vi "RemoteVI App Live Data.vi"() -> ()   [LabVIEW 2020]
doc: "Screen Live Data of RemoteVI Application Example.vi: four simulated channels on the graph Live Data (500 samples each, a new block every 100 ms), their maximum and minimum in Statistics. Pause holds the picture. Runs until the notifier RemoteVI Application Example fires (the main VI quits)."
panel:
  out "Statistics":string[][](table)
  out "Live Data":dbl[][](graph)
  in  "Pause":bool
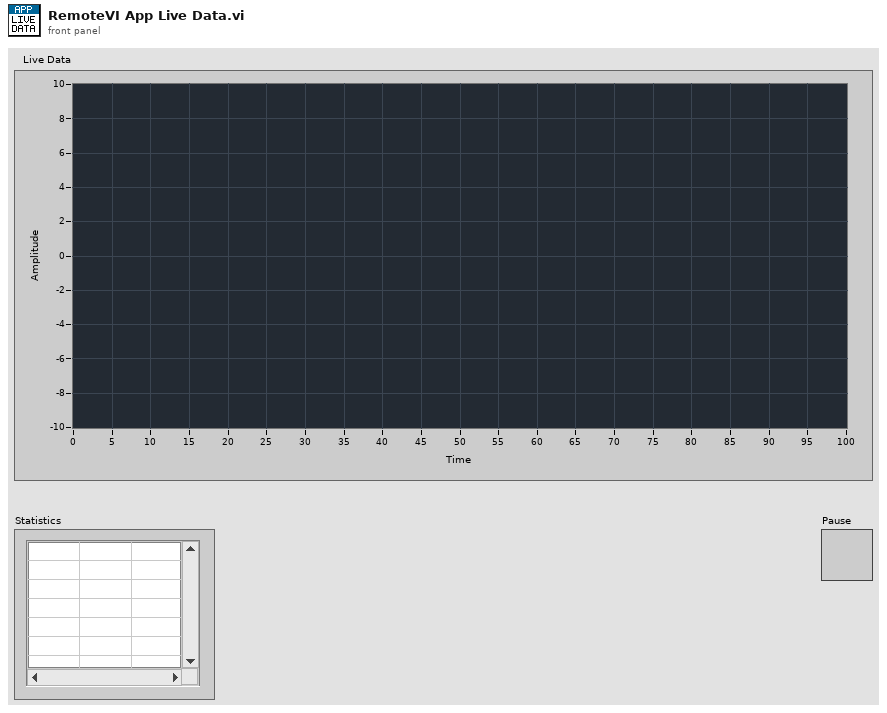
[diagram p1: front panel]
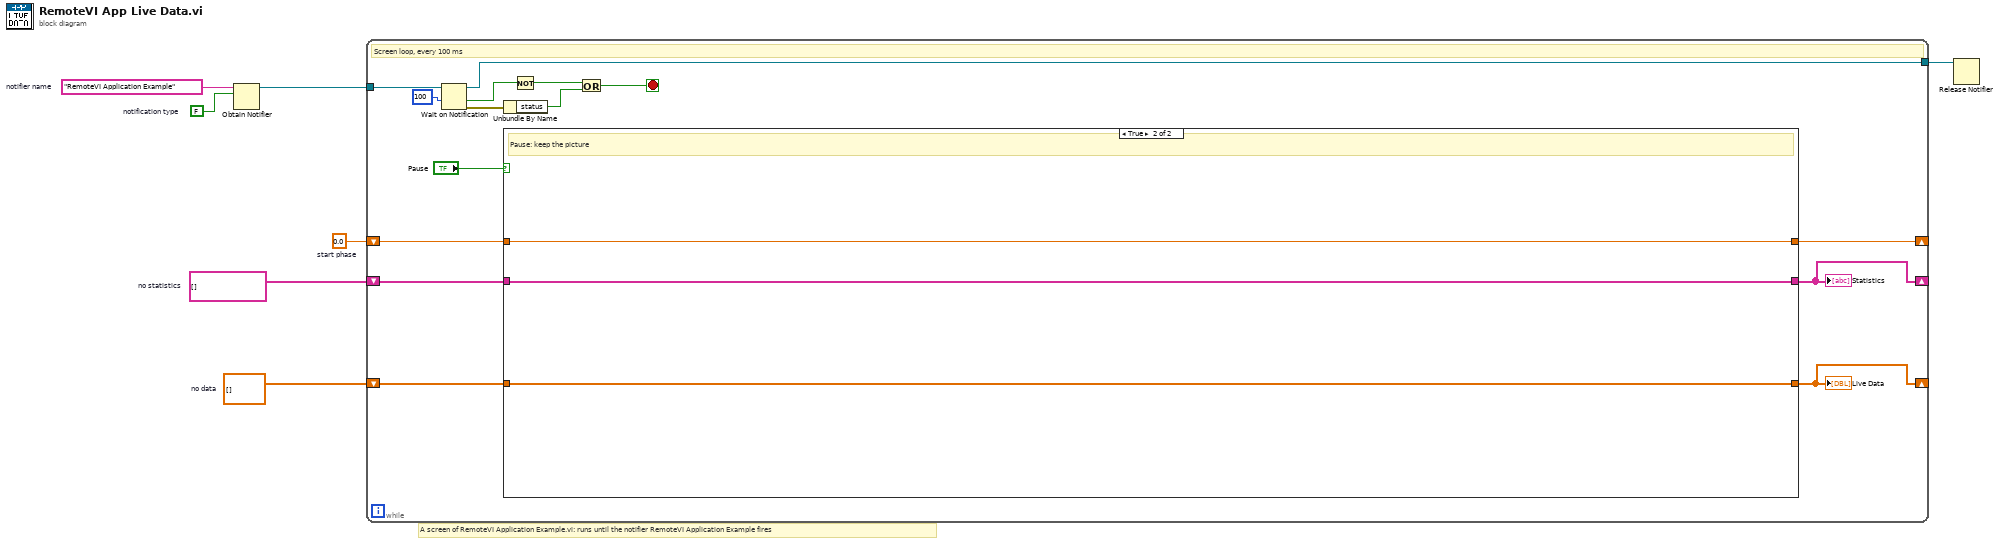
[diagram p0: block diagram]
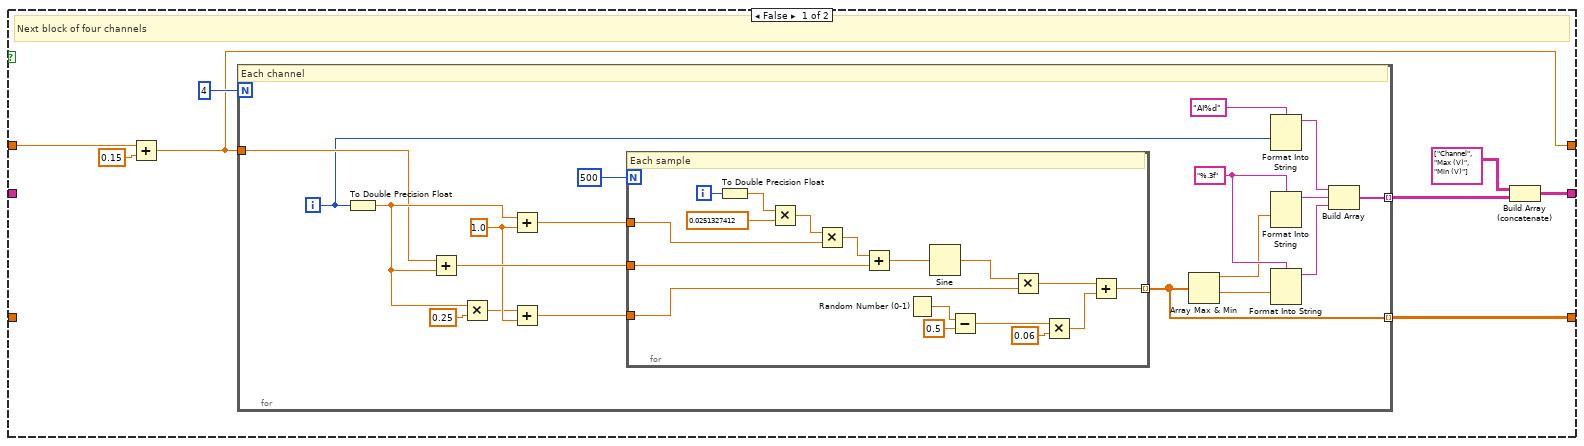
[diagram p2: hidden frame]
diagram:
  w5 = FALSE  # notification type
  w4 = "RemoteVI Application Example"  # notifier name
  w3 = string[][] []  # no statistics
  w2 = dbl[][] []  # no data
  w1 = 0.0  # start phase
  # "A screen of RemoteVI Application Example.vi: runs until the notifier RemoteVI Application Example fires"
  n1 = Obtain Notifier(name (unnamed)=w4, notification data type=w5) -> (notifier out=w6:refnum<notifier>)  [unwired: 2 in, 2 out]
  n2 = while {
    shift-right: [w10] -> _
    shift-left: w1 -> [w9]
    shift-right: [w12] -> _
    shift-left: w2 -> [w11]
    shift-right: [w14] -> _
    shift-left: w3 -> [w13]
    tunnel: w6 -> [w8]
    tunnel: [w17] -> w7
    stop <- w22 stop-if-true
    # "Screen loop, every 100 ms"
    n3 = Wait on Notification(notifier=w8, timeout in ms (-1)=100) -> (notifier out=w17:refnum<notifier>, timed out?=w18:bool, error out=w19:errorcluster)  [unwired: 2 in, 1 out]
    n4 = Unbundle By Name(w19) -> ("status"=w21:bool)
    n5 = case shown="True" "Pause" {
      tunnel: w9 -> [w23 w67]
      tunnel: w11 -> [_ w68]
      tunnel: w13 -> [_ w69]
      tunnel: [w25 w67] -> w10
      tunnel: [w27 w68] -> w12
      tunnel: [w30 w69] -> w14
      frame False {
        # "Next block of four channels"
        n6 = Add(x=w23, y=0.15) -> (x+y=w25:dbl)
        n7 = for {
          N: 4 -> [_]
          tunnel: w25 -> [w32]
          tunnel: [w41] -> w27 mode=indexing
          tunnel: [w49] -> w28 mode=indexing
          i -> [w31]
          w46 = "%.3f"
          w36 = 1.0
          # "Each channel"
          n8 = To Double Precision Float(number=w31) -> (double precision float=w33:dbl)
          n9 = Add(x=w32, y=w33) -> (x+y=w39:dbl)
          n10 = Multiply(x=w33, y=0.25) -> (x*y=w35:dbl)
          n11 = Add(x=w33, y=w36) -> (x+y=w38:dbl)
          n12 = Add(x=w35, y=w36) -> (x+y=w37:dbl)
          n13 = for {
            N: 500 -> [_]
            tunnel: w38 -> [w52]
            tunnel: w37 -> [w51]
            tunnel: w39 -> [w53]
            tunnel: [w66] -> w41 mode=indexing
            i -> [w50]
            # "Each sample"
            n14 = To Double Precision Float(number=w50) -> (double precision float=w54:dbl)
            n15 = Multiply(x=w54, y=0.0251327412) -> (x*y=w56:dbl)
            n16 = Multiply(x=w56, y=w52) -> (x*y=w57:dbl)
            n17 = Add(x=w57, y=w53) -> (x+y=w58:dbl)
            n18 = Random Number (0-1)() -> (number: 0 to 1=w61:dbl)
            n19 = Sine(x=w58) -> (sin(x)=w59:dbl)
            n20 = Subtract(x=w61, y=0.5) -> (x-y=w63:dbl)
            n21 = Multiply(x=w59, y=w51) -> (x*y=w60:dbl)
            n22 = Multiply(x=w63, y=0.06) -> (x*y=w65:dbl)
            n23 = Add(x=w60, y=w65) -> (x+y=w66:dbl)
          }
          n24 = Array Max & Min(array=w41) -> (max value=w42:dbl, min value=w43:dbl)  [unwired: 2 out]
          n25 = Format Into String(format string="AI%d", w31) -> (resulting string=w45:string)  [unwired: 2 in, 1 out]
          n26 = Format Into String(format string=w46, w42) -> (resulting string=w47:string)  [unwired: 2 in, 1 out]
          n27 = Format Into String(format string=w46, w43) -> (resulting string=w48:string)  [unwired: 2 in, 1 out]
          n28 = Build Array(w45, w47, w48) -> (w49:string[])
        }
        n29 = Build Array (concatenate)(string[][] [["Channel", "Max (V)", "Min (V)"]], w28) -> (w30:string[][])
      }
      frame True {
        # "Pause: keep the picture"
      }
    }
    "Live Data" <- w12
    "Statistics" <- w14
    n30 = Not(x=w18) -> (.not. x?=w20:bool)
    n31 = Or(x=w20, y=w21) -> (x .or. y?=w22:bool)
  }
  n32 = Release Notifier(notifier=w7) -> ()  [unwired: 2 in, 3 out]
